vi "Get Call Result.vi"(10 "Response header":string, 11 "Response body in":string) -> (2 "Call Result":string, 3 "Response body out":string)   [LabVIEW 2015, in "NI_AWS_Core.lvlib" / "HTTP Request.lvclass"]
uses:
  HTTP Request.lvclass
  <vilib>/regexp/Match Regular Expression.xnode
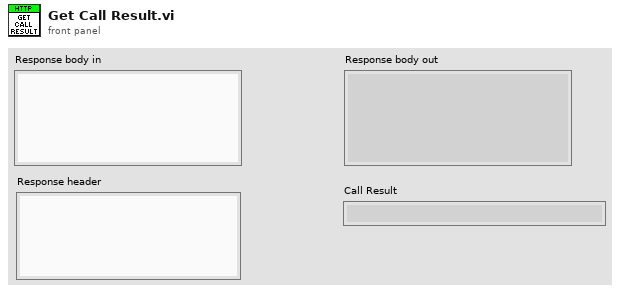
[diagram p1: front panel]
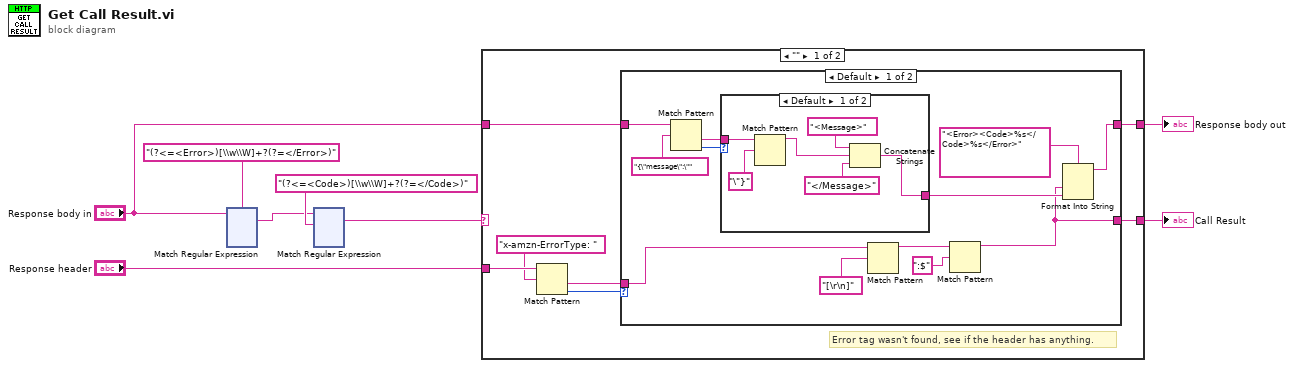
[diagram p0: block diagram]
diagram:
  n1 = xnode "Match Regular Expression"("input string"="Response body in", "regular expression"="(?<=<Error>)[\\w\\W]+?(?=</Error>)") -> ("whole match"=w6:string)  [unwired: 4 in, 4 out]
  n2 = xnode "Match Regular Expression"("input string"=w6, "regular expression"="(?<=<Code>)[\\w\\W]+?(?=</Code>)") -> ("whole match"=w5:string)  [unwired: 4 in, 4 out]
  n3 = case shown="\"\"" w5 {
    selector: w5 -> [_ w36]
    tunnel: [w11 w36] -> w4
    tunnel: "Response header" -> [w15 _]
    tunnel: "Response body in" -> [w10 w35]
    tunnel: [w9 w35] -> w1
    frame "" {
      # "Error tag wasn't found, see if the header has anything."
      n4 = Match Pattern(string=w15, regular expression="x-amzn-ErrorType: ") -> (after substring=w12:string, offset past match=w13:i32)  [unwired: 1 in, 2 out]
      n5 = case shown="Default" w13 {
        tunnel: w12 -> [w27 _]
        tunnel: [w17 _] -> w11
        tunnel: w10 -> [w23 w34]
        tunnel: [w25 w34] -> w9
        frame Default {
          n6 = Match Pattern(string=w23, regular expression="{\"message\":\"") -> (after substring=w20:string, offset past match=w21:i32)  [unwired: 1 in, 2 out]
          n7 = case shown="Default" w21 {
            tunnel: w20 -> [w33 _]
            tunnel: [w28 _] -> w19
            frame Default {
              n8 = Match Pattern(string=w33, regular expression="\"}") -> (before substring=w31:string)  [unwired: 1 in, 3 out]
              n9 = Concatenate Strings("<Message>", w31, "</Message>") -> (w28:string)
            }
            frame -1 {
            }
          }
          n10 = Match Pattern(string=w27, regular expression="[\r\n]") -> (before substring=w18:string)  [unwired: 1 in, 3 out]
          n11 = Match Pattern(string=w18, regular expression=":$") -> (before substring=w17:string)  [unwired: 1 in, 3 out]
          n12 = Format Into String(format string="<Error><Code>%s</Code>%s</Error>", w17, w19) -> (resulting string=w25:string)  [unwired: 2 in, 1 out]
        }
        frame -1 {
        }
      }
    }
    frame Default {
      # "<Error> tag was found, use that."
    }
  }
  "Call Result" <- w4
  "Response body out" <- w1
